vi "Example - Interactive MQTT Client.vi"() -> ()   [LabVIEW 2019]
uses:
  subvis/HMI-States.ctl
  src/KoRE-MQTT.lvlib
  src/KoRE-MQTT/Public/TypeDefs/MQTT Property - Will.ctl
  src/KoRE-MQTT/Public/TypeDefs/MQTT Property - CONNECT.ctl
  src/KoRE-MQTT/Private/TypeDefs/MQTT Subscription - Info.ctl
  src/KoRE-MQTT/Public/TypeDefs/MQTT Client Session - Data.ctl
panel:
  out "mqtt ref data":T1={"TCP ref"=refnum, "Next Packet Id"=0, "Version"=0, "Host"="localhost", "Port"=1883, "Ping Delta"=60, "Username"="", "Password"="", "Will QoS"=0, "Will Retain"=FALSE, "Will Topic"="", "Will Payload"="", "TCP Timeout"=1000, "Semaphore"=refnum, "In-Flight Messages"=variant, "Close"=FALSE, "Last Send"=0, "Keep Alive"=0, "Last Ping RTT"=0, "Last Ping"=0, "Will Properties"=[], "Session Expiry Interval"=0, "Maximum QoS"=0, "Retain Available"=FALSE, "Server Maximum Packet Size"=0, "Client Identifier"="", "Server Topic Alias Maximum"=0, "Wildcard Subscription Available"=FALSE, "Subscription Identifier Available"=FALSE, "Shared Subscription Available"=FALSE, "Connect Properties"=[], "Client Maximum Packet Size"=0, "Client Topic Alias Maximum"=0, "Server Receive Maximum"=0, "Client Receive Maximum"=0, "TLS cfg"=refnum, "Subscriptions"=[]} {"Connect Properties"."Property" items=[" Session Expiry Interval           "=17, " Authentication Method             "=21, " Authentication Data               "=22, " Request Problem Information       "=23, " Request Response Information      "=25, " Receive Maximum                   "=33, " Topic Alias Maximum               "=34, " User Property                     "=38, " Maximum Packet Size               "=39]; "Will Properties"."Property" items=[" Payload Format Indicator          "=1, " Message Expiry Interval           "=2, " Content Type                      "=3, " Response Topic                    "=8, " Correlation Data                  "=9, " Will Delay Interval               "=24, " User Property                     "=38]}
  in  "debug slowdown":u32
  in  "QoS":enum16{"0", "1", "2"}(ring)
  in  "Clean Start":bool
  out "Last error":string
  in  "TLS":bool
  in  "QoS Level":T6(ring)
  in  "Retain":bool
  in  "Topic":string
  in  "Publish":bool
  in  "Message":string
  out "Reconnect errors":i32
  in  "Password":string
  in  "Client ID":string
  in  "Port":u16=1883
  in  "Host":string(combo)="test.mosquitto.org"
  in  "Username":string
  in  "Version":u16(ring)=5 items=["3.11"=4, "5.0"=5]
  out "Messages":u64
  in  "Exit":bool
  in  "Topic filter":string(combo)
  in  "Subscriptions":i32[](listbox)
  in  "Unsubscribe":bool
  in  "Subscribe":bool
  in  "Reconnect":bool
  in  "Disconnect":bool
  in  "Connect":bool
  in  "Tree":string(tree)
  # "-------------------------------------------------------- SCROLL DOWN TO SEE INTERNAL SESSION INFORMATION ---------------------------------------------------"
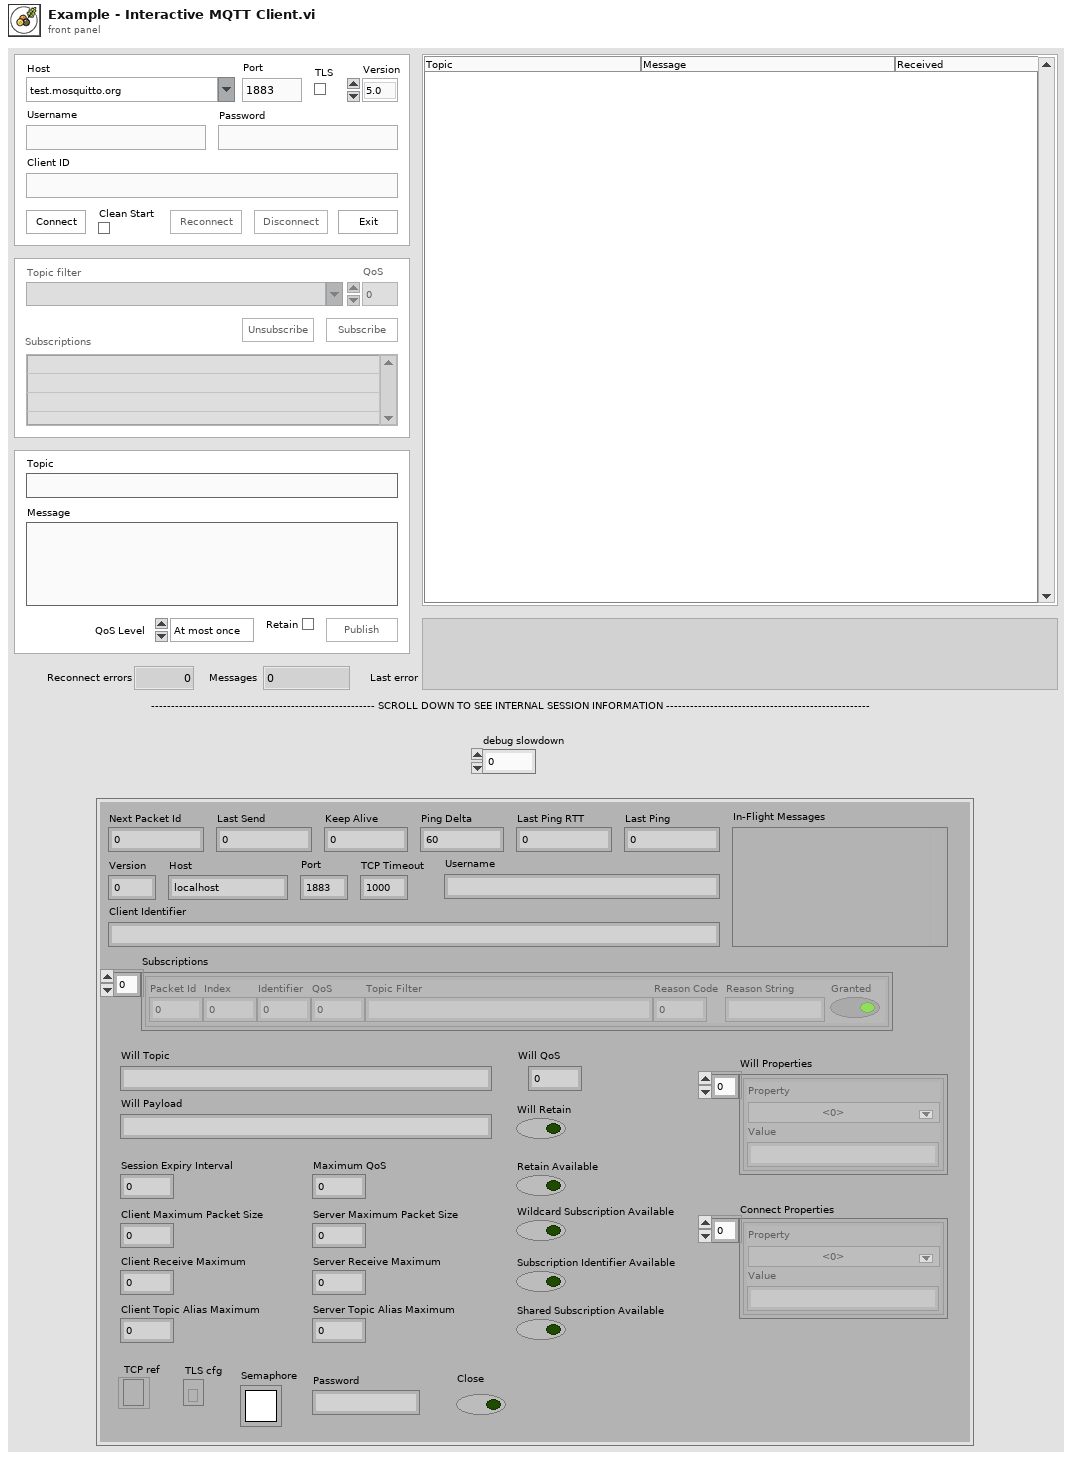
[diagram p1: front panel]
types:
  T1 = typedef "KoRE-MQTT.lvlib/MQTT Client Session - Data.ctl" = cluster{"TCP ref":refnum<k5>, "Next Packet Id":u16, "Version":u8, "Host":string, "Port":u16, "Ping Delta":u32, "Username":string, "Password":string, "Will QoS":u8, "Will Retain":bool, "Will Topic":string, "Will Payload":string, "TCP Timeout":i32, "Semaphore":T2, "In-Flight Messages":variant, "Close":bool, "Last Send":u32, "Keep Alive":u16, "Last Ping RTT":u32, "Last Ping":u32, "Will Properties":T3[], "Session Expiry Interval":u32, "Maximum QoS":u8, "Retain Available":bool, "Server Maximum Packet Size":u32, "Client Identifier":string, "Server Topic Alias Maximum":u16, "Wildcard Subscription Available":bool, "Subscription Identifier Available":bool, "Shared Subscription Available":bool, "Connect Properties":T4[], "Client Maximum Packet Size":u32, "Client Topic Alias Maximum":u16, "Server Receive Maximum":u16, "Client Receive Maximum":u16, "TLS cfg":refnum<k36>, "Subscriptions":T5[]}
  T2 = typedef "Semaphore RefNum" = refnum<k1>
  T3 = typedef "KoRE-MQTT.lvlib/MQTT Property - Will.ctl" = cluster{"Property":u8, "Value":string}
  T4 = typedef "KoRE-MQTT.lvlib/MQTT Property - CONNECT.ctl" = cluster{"Property":u8, "Value":string}
  T5 = typedef "KoRE-MQTT.lvlib/MQTT Subscription - Info.ctl" = cluster{"Packet Id":u16, "Index":u16, "Identifier":u32, "QoS":u8, "Topic Filter":string, "Reason Code":u8, "Reason String":string, "Granted":bool}
  T6 = enum16{"At most once", "At least once", "Exactly once"}
  T7 = typedef "HMI-States.ctl" = enum16{"Noop", "Initialize", "Connect", "Reconnect", "Subscribe", "Publish", "Unsubscribe", "Disconnect", "Exit", "8", "9", "10", "11", "12", "13", "14", "15", "16", "17", "18", "19", "Idle", "Connected"}
  T8 = typedef "KoRE-MQTT.lvlib/MQTT Client Session.ctl" = refnum<vi>
  T9 = enum8{"Enabled", "Disabled", "Disabled and Grayed Out"}
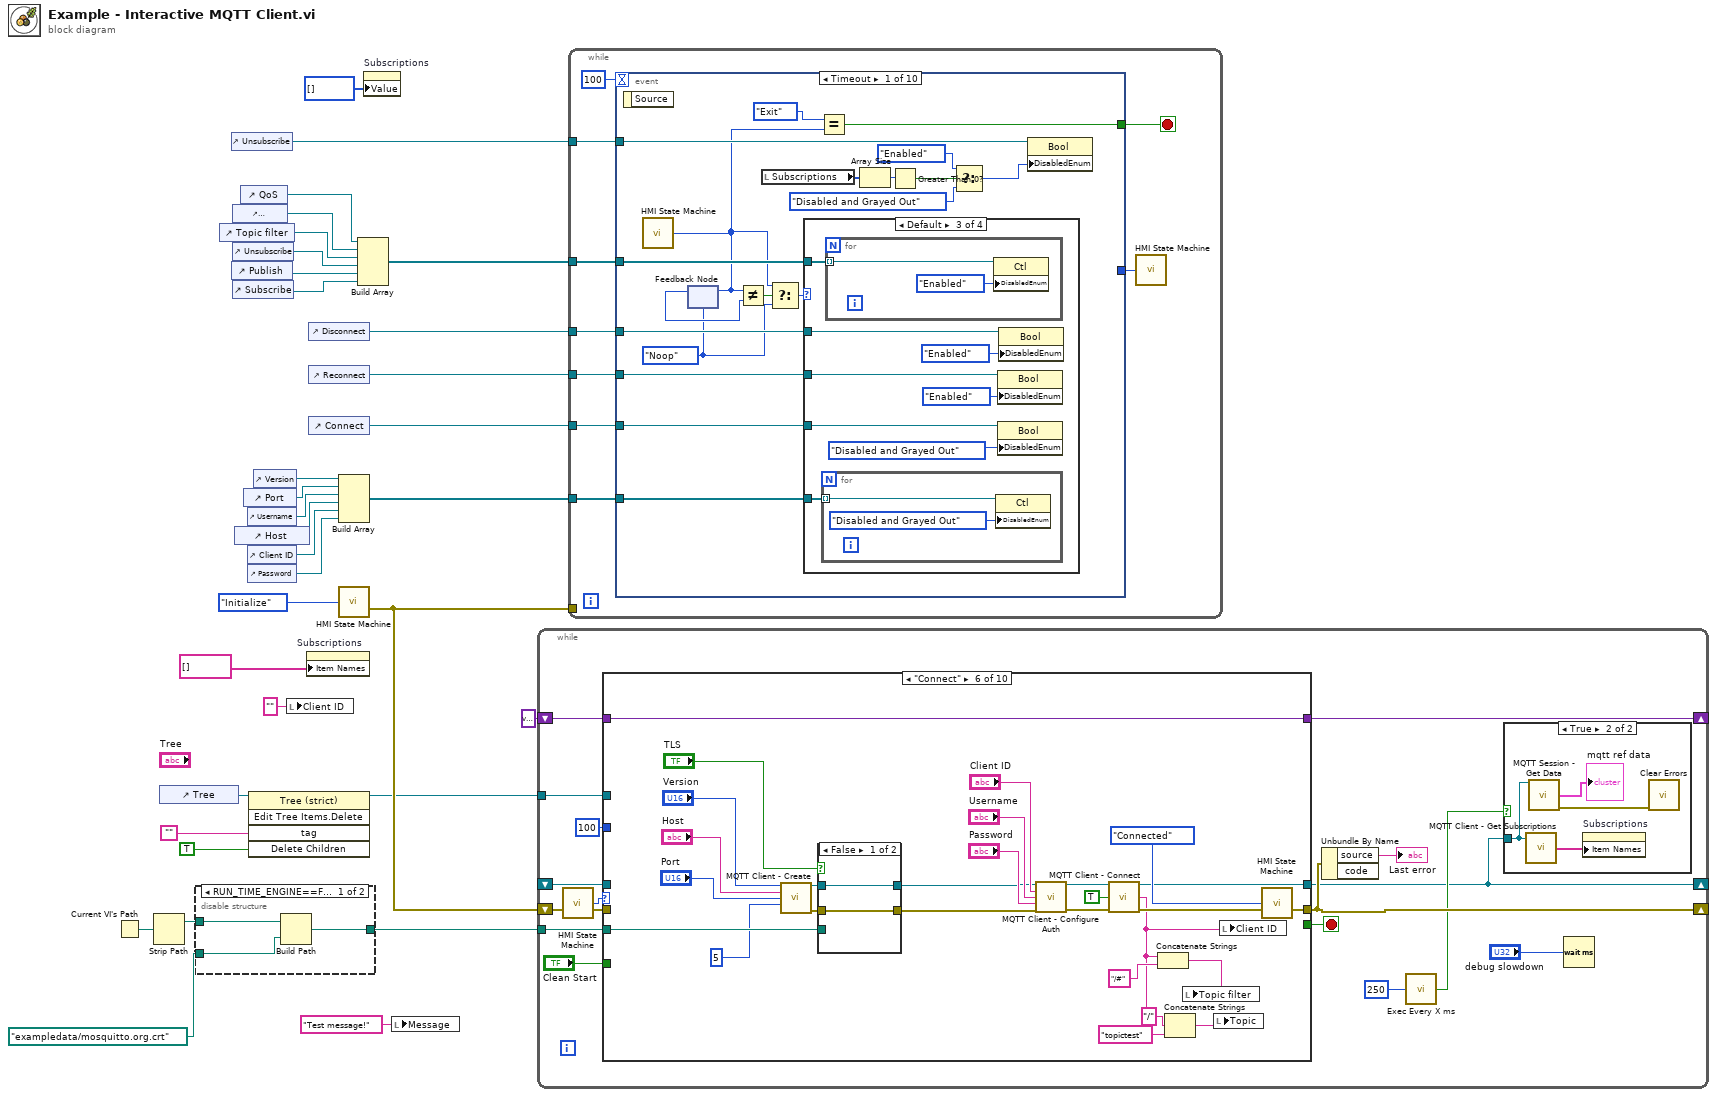
[diagram p0: block diagram]
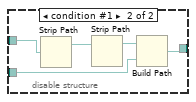
[diagram p2: hidden frame]
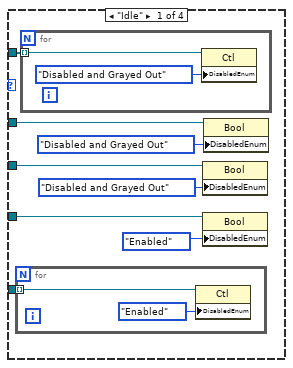
[diagram p3: hidden frame]
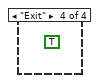
[diagram p5: hidden frame]
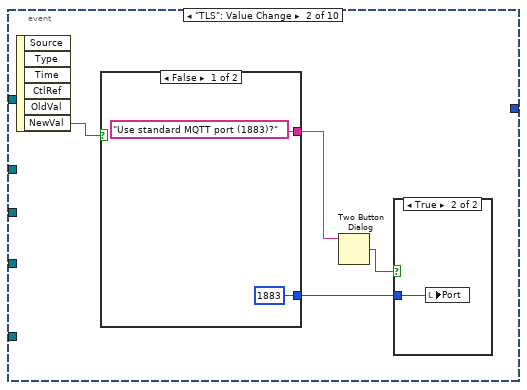
[diagram p6: hidden frame]
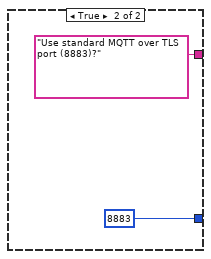
[diagram p8: hidden frame]
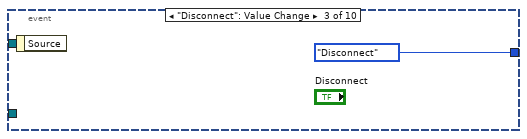
[diagram p9: hidden frame]
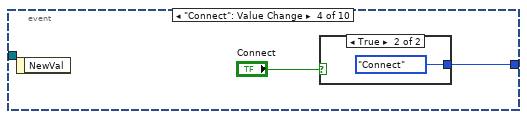
[diagram p10: hidden frame]
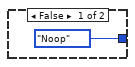
[diagram p11: hidden frame]
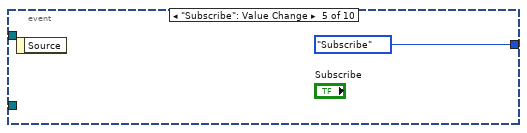
[diagram p12: hidden frame]
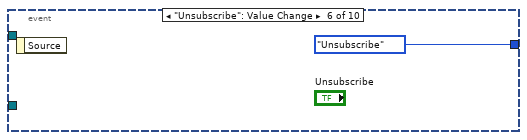
[diagram p13: hidden frame]
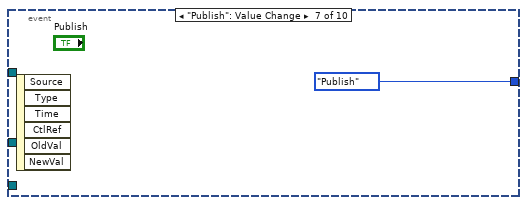
[diagram p14: hidden frame]
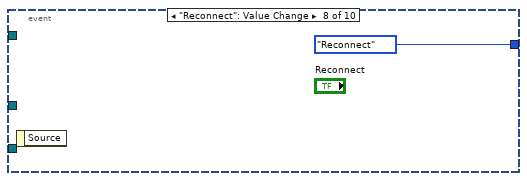
[diagram p15: hidden frame]
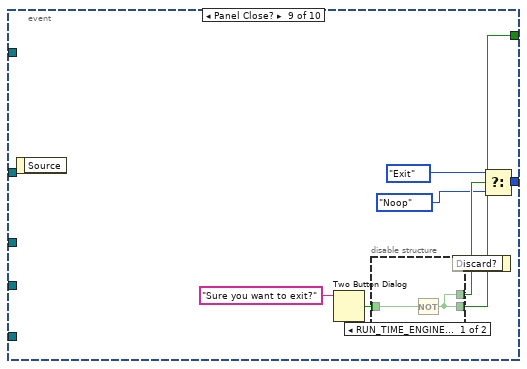
[diagram p16: hidden frame]
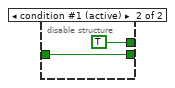
[diagram p17: hidden frame]
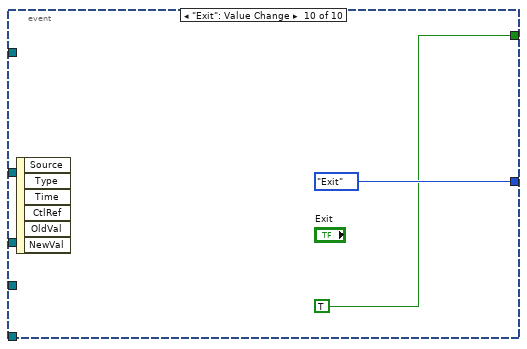
[diagram p18: hidden frame]
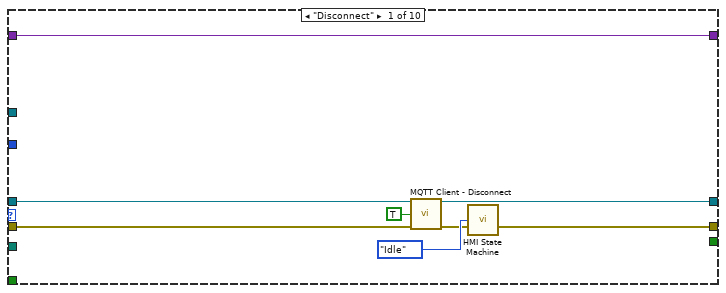
[diagram p20: hidden frame]
diagram:
  n1 = Current VI's Path() -> (path=w6:path)
  n2 = Strip Path(path=w6) -> (stripped path=w5:path)  [unwired: 1 out]
  n3 = control-ref of="Tree"() -> (w12:refnum<vi>)
  n4 = disable-structure shown="RUN_TIME_ENGINE==False" {
    disable-tunnel: w5 -> [w36 w38]
    disable-tunnel: path "exampledata/mosquitto.org.crt" ("name or relative path") -> [w35 w40]
    disable-tunnel: [w34 w41] -> w3
    frame condition #0 (active) {
      n5 = Build Path(base path=w36, name or relative path=w35) -> (appended path=w34:path)
    }
    frame condition #1 {
      n6 = Strip Path(path=w38) -> (stripped path=w37:path)  [unwired: 1 out]
      n7 = Strip Path(path=w37) -> (stripped path=w39:path)  [unwired: 1 out]
      n8 = Build Path(base path=w39, name or relative path=w40) -> (appended path=w41:path)
    }
  }
  n9 = control-ref of="Topic filter"() -> (w29:refnum<vi>)
  n10 = control-ref of="Unsubscribe"() -> (w8:refnum<vi>)
  n11 = control-ref of="Publish"() -> (w10:refnum<vi>)
  n12 = control-ref of="Subscriptions"() -> (w30:refnum<vi>)
  n13 = control-ref of="Unsubscribe"() -> (w27:refnum<vi>)
  n14 = control-ref of="Subscribe"() -> (w28:refnum<vi>)
  n15 = control-ref of="Host"() -> (w17:refnum<vi>)
  n16 = control-ref of="QoS"() -> (w1:refnum<vi>)
  n17 = control-ref of="Port"() -> (w19:refnum<vi>)
  n18 = control-ref of="Username"() -> (w18:refnum<vi>)
  n19 = control-ref of="Client ID"() -> (w11:refnum<vi>)
  n20 = control-ref of="Password"() -> (w16:refnum<vi>)
  n21 = invoke class="Tree (strict)" method="Edit Tree Items.Delete"(reference=w12, "tag"="", "Delete Children"=TRUE ("Delete Children?")) -> (reference out=w13:refnum<vi>)  [unwired: 2 in, 4 out]
  n22 = control-ref of="Version"() -> (w20:refnum<vi>)
  n23 = local write "Client ID"("" ("Client ID")) -> ()
  n24 = property on="Subscriptions" class="LstBox (strict)"("Item Names"=string[] []) -> ()  [unwired: 2 in, 2 out]
  n25 = control-ref of="Disconnect"() -> (w23:refnum<vi>)
  n26 = control-ref of="Reconnect"() -> (w24:refnum<vi>)
  n27 = control-ref of="Connect"() -> (w25:refnum<vi>)
  n28 = Build Array(w20, w19, w18, w17, w11, w16) -> (w22:refnum<vi>[])
  n29 = call "HMI State Machine.vi"("Get/Set State"=HMI-States."Initialize") -> ("error out"=w31:errorcluster)  [unwired: 13 in, 1 out]
  n30 = Build Array(w1, w30, w29, w27, w10, w28) -> (w26:refnum<vi>[])
  n31 = property on="Subscriptions" class="LstBox (strict)"("Value"=i32[] [] ("Subscriptions")) -> ()  [unwired: 2 in, 2 out]
  n32 = local write "Message"("Test message!" ("Message")) -> ()
  n33 = while {
    shift-right: [w51] -> _
    shift-left: w31 -> [w53]
    shift-right: [w42] -> _
    shift-left: _ -> [w58]
    shift-right: [w48] -> _
    shift-left: variant ("Empty Cluster") -> [w57]
    tunnel: w13 -> [w52]
    tunnel: w3 -> [w49]
    stop <- w56 stop-if-true
    n34 = call "HMI State Machine.vi"("error in (no error)"=w53) -> ("State"=w55:T7, "error out"=w54:errorcluster)  [unwired: 13 in]
    n35 = case shown="\"Connect\"" w55 {
      tunnel: w58 -> [w67 w83 w113 w122 w131 _ w181 w192 w216 w219]
      tunnel: [w65 w81 w112 w122 w129 w156 w184 w194 w216 w219] -> w42
      tunnel: w54 -> [w66 w82 w115 w121 w130 _ w180 w191 w215 w218]
      tunnel: [w69 w72 w116 w121 w132 w158 w186 w196 w215 w218] -> w51
      tunnel: [w63 w77 w118 w120 w134 w157 w185 w197 w214 w217] -> w48
      tunnel: w57 -> [w63 w74 w118 w120 w134 w157 w185 w197 w214 w217]
      tunnel: [_ _ _ _ _ _ _ _ TRUE _] -> w56
      tunnel: w52 -> [_ w75 _ _ _ _ _ _ _ _]
      tunnel: 100 -> [_ w71 _ w119 _ _ _ _ _ _]
      tunnel: w49 -> [_ _ _ _ _ w145 _ _ _ _]
      tunnel: "Clean Start" -> [_ _ _ _ _ _ w179 _ _ _]
      frame "Disconnect" {
        n36 = call "MQTT Client - Disconnect.vi"("MQTT Session"=w67, "With Will (v5)"=TRUE ("With Will"), "error in (no error)"=w66) -> ("MQTT Session out"=w65:T8, "error out"=w64:errorcluster)  [unwired: 11 in]
        n37 = call "HMI State Machine.vi"("Get/Set State"=HMI-States."Idle", "error in (no error)"=w64) -> ("error out"=w69:errorcluster)  [unwired: 12 in, 1 out]
      }
      frame "Connected" {
        n38 = call "MQTT Client - Read.vi"("MQTT Session"=w83, "timeout (global)"=w71, "error in (no error)"=w82) -> ("# received"=→"Messages":u64, "MQTT Session out"=w81:T8, "Topic"=w78:string, "Message"=w79:string, "New message?"=w80:bool, "error out"=w73:errorcluster)  [unwired: 6 in, 1 out]
        n39 = case shown="Error .." w73 {
          selector: w73 -> [w84 _]
          tunnel: [w84 w93] -> w72
          frame No Error {
          }
          frame Error {
            n40 = feedback #1() -> (w92:i32)  [unwired: 1 in]
            n41 = Add(x=w92, y=1) -> (x+y=w90:i32)
            "Reconnect errors" <- w90
            n42 = feedback-in #1(w90) -> ()
            n43 = for {
              N: 20 -> [_]
              tunnel: [w96] -> w89
              tunnel: [w94] -> w85
              stop <- w96 continue-if-true
              n44 = call "HMI State Machine.vi"() -> ("State"=w94:T7)  [unwired: 14 in, 1 out]
              n45 = Equal?(x=HMI-States."Connected" ("Get/Set State"), y=w94) -> (x = y?=w96:bool)
              n46 = Wait (ms)(milliseconds to wait=u32 100) -> ()  [unwired: 1 out]
            }
            n47 = Select(t=HMI-States."Reconnect" ("Get/Set State"), s=w89, f=w85) -> (s? t:f=w87:T7)
            n48 = call "HMI State Machine.vi"("Get/Set State"=w87) -> ("error out"=w93:errorcluster)  [unwired: 13 in, 1 out]
          }
        }
        n49 = case shown="False" w80 {
          tunnel: w78 -> [_ w102]
          tunnel: w79 -> [_ w101]
          tunnel: [w98 w99] -> w77
          tunnel: w74 -> [w98 w107]
          tunnel: w75 -> [_ w100]
          frame False {
          }
          frame True {
            n50 = Set Variant Attribute(Variant=w107, name=w102, value=w101) -> (Variant out=w99:variant, error out=w106:errorcluster)  [unwired: 1 in, 1 out]
            n51 = Format Date/Time String(time format string (%c)="%y-%m-%dT%H:%M:%S%3uZ") -> (date/time string=w104:string)  [unwired: 2 in]
            n52 = call <vilib>:"Clear Errors.vi"("error in (no error)"=w106) -> ()  [unwired: 5 in, 2 out]
            n53 = Build Array(w101, w104) -> (w105:string[])
            n54 = call "Insert Into TreeView.vi"("Item values"=w105, "Item path"=w102, "TreeControl Ref"=w100) -> ()  [unwired: 7 in, 2 out]
          }
        }
      }
      frame "Publish" {
        n55 = call "MQTT Client - Publish.vi"("MQTT Session"=w113, "Retain"="Retain", "Topic"="Topic", "Message"="Message", "QoS"="QoS Level", "error in"=w115) -> ("MQTT Session out"=w112:T8, "error out"=w114:errorcluster)  [unwired: 8 in]
        n56 = call "HMI State Machine.vi"("Get/Set State"=HMI-States."Connected", "error in (no error)"=w114) -> ("error out"=w116:errorcluster)  [unwired: 12 in, 1 out]
      }
      frame "Idle" {
        n57 = Wait (ms)(milliseconds to wait=w119) -> ()  [unwired: 1 out]
      }
      frame "Subscribe" {
        n58 = To Unsigned Byte Integer(number="QoS") -> (unsigned 8bit integer=w126:u8)
        n59 = Empty String/Path?(string/path="Topic filter") -> (empty?=w124:bool)
        n60 = Not(x=w124) -> (.not. x?=w123:bool)
        n61 = case shown="True" w123 {
          tunnel: "Topic filter" -> [_ w137]
          tunnel: w131 -> [w136 w141]
          tunnel: w130 -> [w135 _]
          tunnel: [w136 w140] -> w129
          tunnel: [w135 w139] -> w128
          tunnel: w126 -> [_ w138]
          frame False {
          }
          frame True {
            n62 = call "MQTT Client - Subscribe.vi"("MQTT Session"=w141, "Single Topic Filter"=w137, "Single Topic QoS"=w138) -> ("MQTT Session out"=w140:T8, "error out"=w139:errorcluster)  [unwired: 11 in]
            n63 = property on="Topic filter" class="CmbBox"("Value"="" ("Empty String Constant")) -> ()  [unwired: 2 in, 2 out]
          }
        }
        n64 = call "HMI State Machine.vi"("Get/Set State"=HMI-States."Connected", "error in (no error)"=w128) -> ("error out"=w132:errorcluster)  [unwired: 12 in, 1 out]
      }
      frame "Connect" {
        n65 = call "MQTT Client - Create.vi"("Version (3.11)"="Version", "Host"="Host", "Port (1883)"="Port", "Keep Alive (60 s)"=u16 5) -> ("MQTT Session"=w168:T8, "error out"=w148:errorcluster)  [unwired: 10 in]
        n66 = case shown="False" "TLS" {
          tunnel: w168 -> [w171 w176]
          tunnel: [w171 w175] -> w149
          tunnel: w148 -> [w170 w174]
          tunnel: [w170 w173] -> w147
          tunnel: w145 -> [_ w172]
          frame False {
          }
          frame True {
            n67 = call "MQTT Client - Configure TLS.vi"("MQTT Session"=w176, "error in (no error)"=w174, "Trusted Certificates (PEM)"=w172) -> ("MQTT Session out"=w175:T8, "error out"=w173:errorcluster)  [unwired: 11 in]
          }
        }
        n68 = call "MQTT Client - Configure Auth.vi"("MQTT Session"=w149, "Client ID"="Client ID", "Username"="Username", "Password"="Password", "error in (no error)"=w147) -> ("MQTT Session out"=w161:T8, "error out"=w160:errorcluster)  [unwired: 9 in]
        n69 = call "MQTT Client - Connect.vi"("MQTT Session"=w161, "Clean Start"=TRUE, "error in (no error)"=w160) -> ("MQTT Session out"=w156:T8, "Assigned Client Identifier"=w150:string, "error out"=w159:errorcluster)  [unwired: 8 in, 2 out]
        n70 = Concatenate Strings(w150, "/#" ("string")) -> (w154:string)
        n71 = Concatenate Strings(w150, "/" ("string"), "topictest" ("string")) -> (w155:string)
        n72 = local write "Topic filter"(w154) -> ()
        n73 = local write "Topic"(w155) -> ()
        n74 = local write "Client ID"(w150) -> ()
        n75 = call "HMI State Machine.vi"("Get/Set State"=HMI-States."Connected", "error in (no error)"=w159) -> ("error out"=w158:errorcluster)  [unwired: 12 in, 1 out]
      }
      frame "Reconnect" {
        n76 = call "MQTT Client - Disconnect.vi"("MQTT Session"=w181, "With Will (v5)"=TRUE ("With Will"), "error in (no error)"=w180) -> ("MQTT Session out"=w178:T8, "error out"=w177:errorcluster)  [unwired: 11 in]
        n77 = call "MQTT Client - Connect.vi"("MQTT Session"=w178, "Clean Start"=w179, "error in (no error)"=w177) -> ("MQTT Session out"=w184:T8, "Assigned Client Identifier"=w183:string, "error out"=w187:errorcluster)  [unwired: 8 in, 2 out]
        n78 = local write "Client ID"(w183) -> ()
        n79 = call "HMI State Machine.vi"("Get/Set State"=HMI-States."Connected", "error in (no error)"=w187) -> ("error out"=w186:errorcluster)  [unwired: 12 in, 1 out]
      }
      frame "Unsubscribe" {
        n80 = Array Size(array="Subscriptions") -> (size(s)=w190:i32)
        n81 = Greater Than 0?(x=w190) -> (x > 0?=w198:bool)
        n82 = case shown="True" w198 {
          tunnel: "Subscriptions" -> [_ w202]
          tunnel: [w200 w207] -> w194
          tunnel: [w199 w206] -> w193
          tunnel: w192 -> [w200 w205]
          tunnel: w191 -> [w199 w204]
          frame False {
          }
          frame True {
            n83 = property on="Subscriptions" class="LstBox (strict)"() -> ("Item Names"=w203:string[])  [unwired: 2 in, 2 out]
            n84 = for {
              tunnel: w203 -> [w212] mode=indexing
              tunnel: w202 -> [w210]
              tunnel: [w212] -> w201 mode=indexing if=w208
              workers-P: _ -> [_]
              i -> [w211]
              n85 = Search 1D Array(1D array=w210, element=w211) -> (index of element=w209:i32)  [unwired: 1 in]
              n86 = Greater Or Equal To 0?(x=w209) -> (x >= 0?=w208:bool)
            }
            n87 = call "MQTT Client - Unsubscribe.vi"("MQTT Session"=w205, "Topic Filters"=w201, "error in (no error)"=w204) -> ("MQTT Session out"=w207:T8, "error out"=w206:errorcluster)  [unwired: 11 in]
          }
        }
        n88 = call "HMI State Machine.vi"("Get/Set State"=HMI-States."Connected", "error in (no error)"=w193) -> ("error out"=w196:errorcluster)  [unwired: 12 in, 1 out]
      }
      frame "Exit" {
      }
      frame Default {
      }
    }
    n89 = Unbundle By Name(w51) -> ("source"=→"Last error":string)  [unwired: 1 out]
    n90 = call "Exec Every X ms.vi"("Trigger interval (1000ms)"=u32 250) -> ("Trigged?"=w43:bool)  [unwired: 4 in]
    n91 = case shown="True" w43 {
      tunnel: w42 -> [_ w59]
      frame False {
      }
      frame True {
        n92 = call "MQTT Client - Get Subscriptions.vi"("MQTT_Q In in"=w59) -> ("Topic Filters"=w62:string[])  [unwired: 13 in, 1 out]
        n93 = call "MQTT Session - Get Data.vi"("mqtt ref in"=w59) -> ("mqtt ref data"=→"mqtt ref data":T1, "error out"=w61:errorcluster)  [unwired: 12 in, 1 out]
        n94 = property on="Subscriptions" class="LstBox (strict)"("Item Names"=w62) -> ()  [unwired: 2 in, 2 out]
        n95 = call <vilib>:"Clear Errors.vi"("error in (no error)"=w61) -> ()  [unwired: 5 in, 2 out]
      }
    }
    n96 = Wait (ms)(milliseconds to wait="debug slowdown") -> ()  [unwired: 1 out]
  }
  n97 = while {
    tunnel: w31 -> [_]
    tunnel: w26 -> [w221]
    tunnel: w25 -> [w223]
    tunnel: w24 -> [w224]
    tunnel: w23 -> [w225]
    tunnel: w22 -> [w222]
    tunnel: w8 -> [w220]
    stop <- w228 stop-if-true
    n98 = event shown="[0] Timeout" {
      selector: _ -> [_ _ _ _ _ _ _ _ _ _]
      dyn-events: _ -> [_ _ _ _ _ _ _ _ _ _]
      timeout: 100 -> [_ _ _ _ _ _ _ _ _ _]
      tunnel: [w229 _ _ _ _ _ _ _ w294 TRUE ("T button?")] -> w228
      tunnel: [_ _ HMI-States."Disconnect" ("f") w283 HMI-States."Subscribe" ("f") HMI-States."Unsubscribe" ("f") HMI-States."Publish" ("f") HMI-States."Reconnect" w290 HMI-States."Exit" ("f")] -> w227
      tunnel: w225 -> [w247 _ _ _ _ _ _ _ _ _]
      tunnel: w224 -> [w246 _ _ _ _ _ _ _ _ _]
      tunnel: w223 -> [w245 _ _ _ _ _ _ _ _ _]
      tunnel: w222 -> [w244 _ _ _ _ _ _ _ _ _]
      tunnel: w221 -> [w243 _ _ _ _ _ _ _ _ _]
      tunnel: w220 -> [w236 _ _ _ _ _ _ _ _ _]
      event Timeout {
        w239 = HMI-States."Noop" ("State")
        n99 = event-data() -> ()  [unwired: 1 in, 1 out]
        n100 = call "HMI State Machine.vi"() -> ("State"=w231:T7)  [unwired: 14 in, 1 out]
        n101 = feedback-in #2(w231) -> ()
        n102 = feedback #2(w239) -> (w242:T7)
        n103 = Not Equal?(x=w231, y=w242) -> (x != y?=w241:bool)
        n104 = local read "Subscriptions"() -> (w237:i32[])
        n105 = Select(t=w231, s=w241, f=w239) -> (s? t:f=w240:T7)
        n106 = case shown="Default" w240 {
          tunnel: w247 -> [w255 _ w267 _]
          tunnel: w246 -> [w254 _ w266 _]
          tunnel: w245 -> [w250 _ w262 _]
          tunnel: w244 -> [w249 _ w261 _]
          tunnel: w243 -> [w248 _ w260 _]
          frame "Idle" {
            n107 = for {
              tunnel: w249 -> [w259] mode=indexing
              n108 = property on="Property Node" class="Ctl"(reference=w259, "DisabledEnum"=T9."Enabled" ("Disabled")) -> ()  [unwired: 1 in, 2 out]
            }
            n109 = for {
              tunnel: w248 -> [w257] mode=indexing
              n110 = property on="Property Node" class="Ctl"(reference=w257, "DisabledEnum"=T9."Disabled and Grayed Out" ("Disabled")) -> ()  [unwired: 1 in, 2 out]
            }
            n111 = property on="Property Node" class="Bool"(reference=w254, "DisabledEnum"=T9."Disabled and Grayed Out" ("Disabled")) -> ()  [unwired: 1 in, 2 out]
            n112 = property on="Property Node" class="Bool"(reference=w250, "DisabledEnum"=T9."Enabled" ("Disabled")) -> ()  [unwired: 1 in, 2 out]
            n113 = property on="Property Node" class="Bool"(reference=w255, "DisabledEnum"=T9."Disabled and Grayed Out" ("Disabled")) -> ()  [unwired: 1 in, 2 out]
          }
          frame "Noop" {
          }
          frame Default {
            n114 = for {
              tunnel: w261 -> [w271] mode=indexing
              n115 = property on="Property Node" class="Ctl"(reference=w271, "DisabledEnum"=T9."Disabled and Grayed Out" ("Disabled")) -> ()  [unwired: 1 in, 2 out]
            }
            n116 = for {
              tunnel: w260 -> [w269] mode=indexing
              n117 = property on="Property Node" class="Ctl"(reference=w269, "DisabledEnum"=T9."Enabled" ("Disabled")) -> ()  [unwired: 1 in, 2 out]
            }
            n118 = property on="Property Node" class="Bool"(reference=w266, "DisabledEnum"=T9."Enabled" ("Disabled")) -> ()  [unwired: 1 in, 2 out]
            n119 = property on="Property Node" class="Bool"(reference=w262, "DisabledEnum"=T9."Disabled and Grayed Out" ("Disabled")) -> ()  [unwired: 1 in, 2 out]
            n120 = property on="Property Node" class="Bool"(reference=w267, "DisabledEnum"=T9."Enabled" ("Disabled")) -> ()  [unwired: 1 in, 2 out]
          }
          frame "Exit" {
            (unwired) TRUE
          }
        }
        n121 = Equal?(x=HMI-States."Exit", y=w231) -> (x = y?=w229:bool)
        n122 = Array Size(array=w237) -> (size(s)=w238:i32)
        n123 = Greater Than 0?(x=w238) -> (x > 0?=w233:bool)
        n124 = Select(t=T9."Enabled" ("Disabled"), s=w233, f=T9."Disabled and Grayed Out" ("Disabled")) -> (s? t:f=w232:T9)
        n125 = property on="Property Node" class="Bool"(reference=w236, "DisabledEnum"=w232) -> ()  [unwired: 1 in, 2 out]
      }
      event "TLS": Value Change {
        n126 = event-data() -> ("NewVal"=w274:bool)  [unwired: 1 in, 5 out]
        n127 = case shown="False" w274 {
          tunnel: ["Use standard MQTT port (1883)?" ("message") "Use standard MQTT over TLS port (8883)?" ("message")] -> w275
          tunnel: [u16 1883 ("Port") u16 8883 ("Port")] -> w272
          frame False {
          }
          frame True {
          }
        }
        n128 = Two Button Dialog(message=w275) -> (T button?=w273:bool)  [unwired: 2 in]
        n129 = case shown="True" w273 {
          tunnel: w272 -> [_ w276]
          frame False {
          }
          frame True {
            n130 = local write "Port"(w276) -> ()
          }
        }
      }
      event "Disconnect": Value Change {
        n131 = event-data() -> ()  [unwired: 1 in, 1 out]
      }
      event "Connect": Value Change {
        n132 = event-data() -> ()  [unwired: 1 in, 1 out]
        n133 = case shown="True" "Connect" {
          tunnel: [HMI-States."Noop" HMI-States."Connect"] -> w283
          frame False {
          }
          frame True {
          }
        }
      }
      event "Subscribe": Value Change {
        n134 = event-data() -> ()  [unwired: 1 in, 1 out]
      }
      event "Unsubscribe": Value Change {
        n135 = event-data() -> ()  [unwired: 1 in, 1 out]
      }
      event "Publish": Value Change {
        n136 = event-data() -> ()  [unwired: 1 in, 6 out]
      }
      event "Reconnect": Value Change {
        n137 = event-data() -> ()  [unwired: 1 in, 1 out]
      }
      event Panel Close? {
        n138 = event-data() -> ()  [unwired: 1 in, 1 out]
        n139 = Two Button Dialog(message="Sure you want to exit?") -> (T button?=w295:bool)  [unwired: 2 in]
        n140 = disable-structure "Conditional Disable Structure" shown="RUN_TIME_ENGINE==True, Default" {
          disable-tunnel: w295 -> [w298 w299]
          disable-tunnel: [w297 TRUE] -> w293
          disable-tunnel: [w297 w299] -> w294
          frame condition #0 {
            n141 = Not(x=w298) -> (.not. x?=w297:bool)
          }
          frame condition #1 (active) {
          }
        }
        n142 = event-data ("Event Filter Node")("Discard?"=w293) -> ()  [unwired: 1 in, 1 out]
        n143 = Select(t=HMI-States."Exit", s=w293, f=HMI-States."Noop") -> (s? t:f=w290:T7)
      }
      event "Exit": Value Change {
        n144 = event-data() -> ()  [unwired: 1 in, 6 out]
      }
    }
    n145 = call "HMI State Machine.vi"("Get/Set State"=w227) -> ()  [unwired: 13 in, 2 out]
  }
